vi "Register gRPC Server.vi"(8 "error in (no error)":errorcluster, 10 "gRPC ID":T1, 11 "CIFPlugin in":refnum<class "CAN_Reader_NIXNET_Plugin.lvclass">) -> (0 "error out":errorcluster, 2 "gRPC ID Out":T1, 3 "CIFPlugin out":refnum<class "CAN_Reader_NIXNET_Plugin.lvclass">)   [LabVIEW 2021, in "CAN_Reader_NIXNET_Plugin.lvclass"]
uses:
  CAN_Reader_NIXNET_Plugin.lvclass
  C:/Program Files/National Instruments/LabVIEW 2021/vi.lib/CIF Foundation/CIF Core/CIFCore/Class/CIFCorePlugin.lvclass
  <vilib>/gRPC/LabVIEW gRPC Library/Shared/grpcId.ctl
  Grpc/CanReaderNixnet_server/RPC Service/CanReaderNixnet/CanReaderNixnet.lvclass
  C:/Program Files/National Instruments/LabVIEW 2021/vi.lib/gRPC/LabVIEW gRPC Servicer/ServiceBase/ServiceBase.lvclass
  <vilib>/CIF Foundation/CIF Core/CIFCore/Class/CIFCorePlugin.lvclass/CIFCorePlugin.ctl
  <vilib>/CIF Foundation/CIF Core/CIFCore/Class/Accessors/Read Register gRPC Descriptors.vi
  <vilib>/gRPC/LabVIEW gRPC Library/Server API/Server/Register Message Metadata.vi
  <vilib>/gRPC/LabVIEW gRPC Library/Server API/Server/Register Enum Metadata.vi
  CAN_Reader_NIXNET_Plugin.lvclass/CAN_Reader_NIXNET_Plugin.ctl
  <vilib>/CIF Foundation/CIF Core/CIFCore/Class/CIFCorePlugin.lvclass
  Grpc/CanReaderNixnet_server/CanReaderNixnet_server.lvlib
  <vilib>/CIF Foundation/CIF U8 Array Monitor gRPC/U8_Array_Monitor_gRPC/CIFU8ArrayMonitorUtilities/CIFU8ArrayMonitorUtilities.lvlib
  <vilib>/gRPC/LabVIEW gRPC Library/grpc-lvsupport-release.lvlib
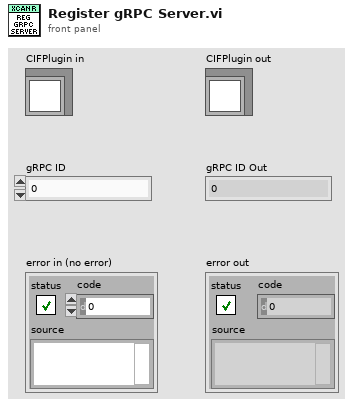
[diagram p1: front panel]
types:
  T1 = typedef "grpc-lvsupport-release.lvlib/grpcId.ctl" = u64
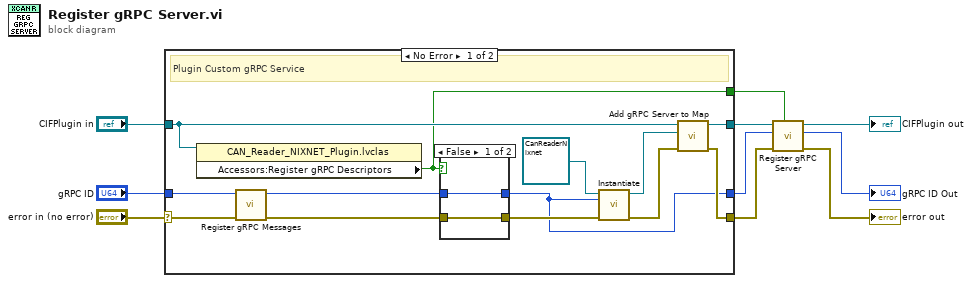
[diagram p0: block diagram]
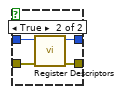
[diagram p2: hidden frame]
diagram:
  n1 = case shown="No Error" "error in (no error)" {
    selector: "error in (no error)" -> [w13 w32]
    tunnel: [w19 w32] -> w5
    tunnel: [w23 w31] -> w7
    tunnel: "CIFPlugin in" -> [w12 w31]
    tunnel: "gRPC ID" -> [w14 w30]
    tunnel: [w15 w30] -> w6
    tunnel: [w11 _] -> w1
    frame No Error {
      # "Plugin Custom gRPC Service"
      n2 = property class="CAN_Reader_NIXNET_Plugin.lvclas"(reference=w12) -> ("Accessors:Register gRPC Descriptors"=w11:bool)  [unwired: 1 in, 2 out]
      n3 = call "Register gRPC Messages.vi"("error in (no error)"=w13, "gRPC ID"=w14) -> ("error out"=w18:errorcluster, "gRPC ID Out"=w17:T1)  [unwired: 8 in]
      n4 = case shown="False" w11 {
        tunnel: w18 -> [w24 w29]
        tunnel: w17 -> [w25 w28]
        tunnel: [w24 w27] -> w16
        tunnel: [w25 w26] -> w15
        frame False {
        }
        frame True {
          n5 = call "Register Descriptors.vi"("error in (no error)"=w29, "gRPC ID"=w28) -> ("error out"=w27:errorcluster, "gRPC ID Out"=w26:T1)  [unwired: 8 in]
        }
      }
      n6 = call-dynamic "Instantiate.vi"("error in"=w16, "gRPCid"=w15, "gRPC service in"=refnum<class "CanReaderNixnet.lvclass"> refnum ("CanReaderNixnet")) -> ("error out"=w21:errorcluster, "gRPC service out"=w20:refnum<class "CanReaderNixnet.lvclass">)  [unwired: 7 in]
      n7 = call <vilib>:"Add gRPC Server to Map.vi"("error in (no error)"=w21, "gRPC Server Class"=w20, "CIFTemplateNode in"=w12) -> ("error out"=w19:errorcluster, "CIFTemplateNode out"=w23:refnum<class "CAN_Reader_NIXNET_Plugin.lvclass">)  [unwired: 7 in]
    }
    frame Error {
    }
  }
  n8 = call <vilib>:"Register gRPC Server.vi"("Register gRPC Descriptors"=w1, "error in"=w5, "gRPC ID"=w6, "CIFNode in"=w7) -> ("error out"=→"error out":errorcluster, "gRPC ID"=→"gRPC ID Out":T1, "CIFNode out"=→"CIFPlugin out":refnum<class "CAN_Reader_NIXNET_Plugin.lvclass">)  [unwired: 5 in]
